vi "Group_Editor.vi"(8 "error in (no error)":errorcluster={"status"=FALSE, "code"=0, "source"="\"\""}, 10 "actions":string, 11 "GroupDefinition":string) -> (0 "error out":errorcluster={"status"=FALSE, "code"=0, "source"="\"\""}, 2 "status ok":bool, 3 "Updated group tree":string)   [LabVIEW 2026]
doc: "INTENT: Define sequential and parallel groups. LOGIC: Create child list, cycles, join policy and resource declarations; show conflicts."
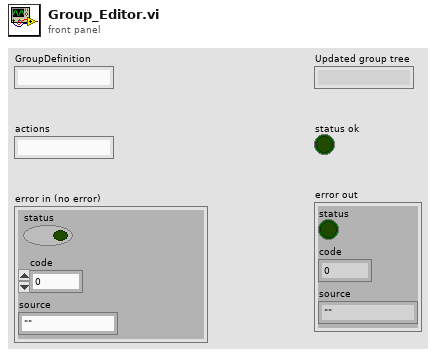
[diagram p1: front panel]
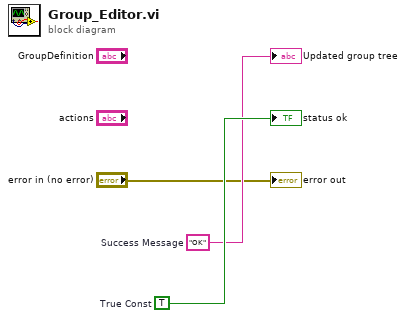
[diagram p0: block diagram]
diagram:
  w3 = TRUE  # True Const
  w2 = "OK"  # Success Message
  "Updated group tree" <- w2
  "status ok" <- w3
  "error out" <- "error in (no error)"
